vi "Main - Run Test Event (eFGV).vi"(7 "Action":T2, 8 "error in":errorcluster, 11 "Data":T1) -> (0 "error out":errorcluster, 2 "Data ref":refnum<user-event>, 3 "Data Out":T1)   [LabVIEW 2019]
uses:
  Controls/eFGV States.ctl
  <vilib>/event_ctls.llb/usereventprio.ctl
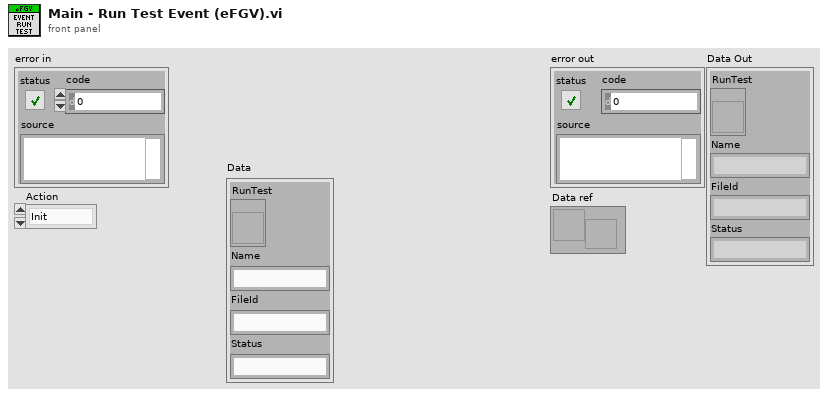
[diagram p1: front panel]
types:
  T1 = cluster{"RunTest":refnum<vi>, "Name":string, "FileId":string, "Status":string}
  T2 = typedef "eFGV States.ctl" = enum16{"Init", "Read", "Write", "Exit"}
  T3 = typedef "usereventprio.ctl" = enum32{"high priority", "normal priority"}
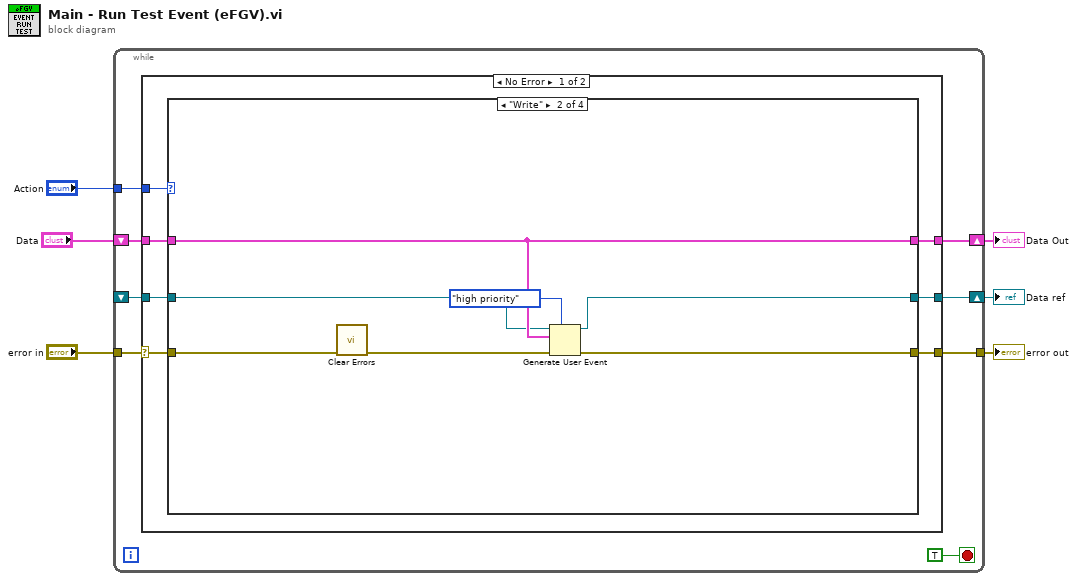
[diagram p0: block diagram]
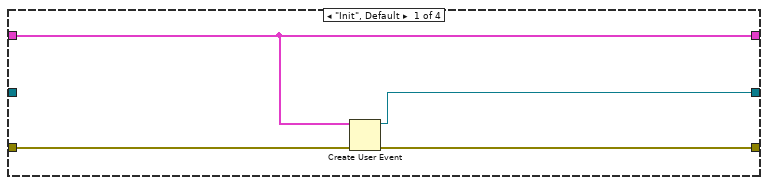
[diagram p2: hidden frame]
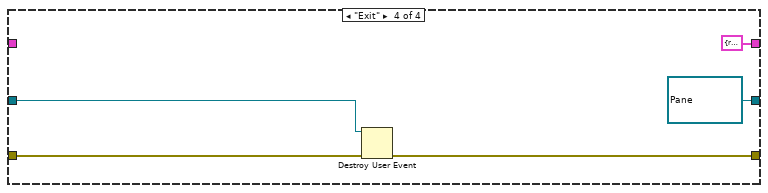
[diagram p4: hidden frame]
diagram:
  n1 = while {
    tunnel: "error in" -> [w13]
    tunnel: [w12] -> w5
    tunnel: "Action" -> [w11]
    shift-right: [w9] -> w2
    shift-left: "Data" -> [w10]
    shift-right: [w8] -> w1
    shift-left: _ -> [w7]
    stop <- TRUE stop-if-true
    n2 = case shown="No Error" w13 {
      selector: w13 -> [w20 w43]
      tunnel: [w21 w43] -> w12
      tunnel: w11 -> [w19 _]
      tunnel: w10 -> [w18 w42]
      tunnel: [w17 w42] -> w9
      tunnel: w7 -> [w16 w41]
      tunnel: [w15 w41] -> w8
      frame No Error {
        n3 = case shown="\"Write\"" w19 {
          tunnel: [w24 w31 w35 w40] -> w21
          tunnel: w20 -> [w25 w30 w35 w39]
          tunnel: w18 -> [w23 w32 w34 _]
          tunnel: [w23 w32 w34 T1 {"RunTest"=refnum, "Name"="", "FileId"="", "Status"=""} ("Data")] -> w17
          tunnel: w16 -> [_ w29 w33 w38]
          tunnel: [w22 w27 w33 refnum<user-event> refnum ("Data")] -> w15
          frame "Init", Default {
            n4 = Create User Event(user event datatype=w23, error in=w25) -> (user event=w22:refnum<user-event>, error out=w24:errorcluster)
          }
          frame "Write" {
            n5 = call <vilib>:"Clear Errors.vi"("error in (no error)"=w30) -> ("error out"=w26:errorcluster)  [unwired: 5 in, 1 out]
            n6 = Generate User Event(priority (normal)=usereventprio."high priority", user event=w29, event data cluster=w32, error in=w26) -> (user event out=w27:refnum<user-event>, error out=w31:errorcluster)
          }
          frame "Read" {
          }
          frame "Exit" {
            n7 = Destroy User Event(user event=w38, error in=w39) -> (error out=w40:errorcluster)
          }
        }
      }
      frame Error {
      }
    }
  }
  "error out" <- w5
  "Data Out" <- w2
  "Data ref" <- w1
